vi "Utility - Build VIHelpeks Help and Link to VIs.vi"() -> ()   [LabVIEW 2014]
doc: "::: VI Helpeks :::\nCopyright (c) 2000-2026 Konstantin Shifershteyn. All rights reserved."
uses:
  <vilib>/Platform/browser.llb/Open URL in Default Browser (path).vi
  vi.lib/addons/VI Helpeks/VIHelpeksAPI.lvlib
panel:
  out "VI Help Info":T1(array[cluster])
  out "error out":errorcluster
  in  "Save Params":T2
  in  "Build Params":T3={"Help Targeting"=enum."<helpdir>", "Subfolder"="VI Helpeks", "CHM Tag mode"=enum."HTML Filename"}
  out "Errors":i32
  out "Paths":T4
  in  "Generate CHM (T)":bool=TRUE
  in  "Show Progress Window (T)":bool=TRUE
  in  "VIHelpeks Project File":path=path "../Help Project/VIHelpeks.hgprj"
  # "VI Helpeks\nCopyright (c) 2012-2026 Konstantin Shifershteyn"
  # "Apply Help Configuration to VIs"
  # "Generate Help"
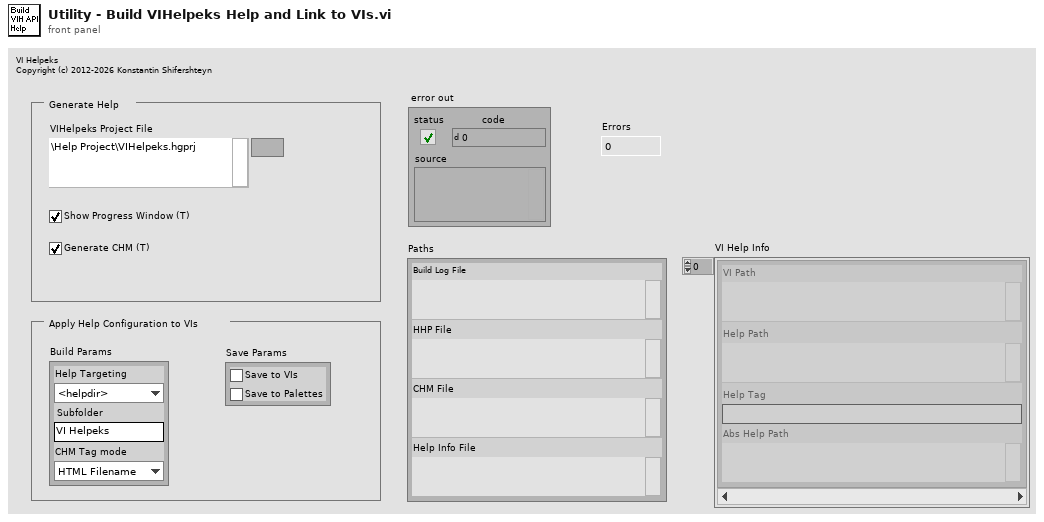
[diagram p1: front panel]
types:
  T1 = cluster{"VI Path":path, "Help Path":path, "Help Tag":string, "Abs Help Path":path}[]
  T2 = cluster{"Save to VIs":bool, "Save to Palettes":bool}
  T3 = cluster{"Help Targeting":enum16{"absolute", "relative", "<helpdir>", "<userlib>", "<vilib>", "<instrlib>"}, "Subfolder":string, "CHM Tag mode":enum16{"HTML Filename", "Index Keyword"}}
  T4 = cluster{"Build Log File":path, "HHP File":path, "CHM File":path, "Help Info File":path}
  T5 = cluster{"Help Path":path, "Help Tag":string, "Abs Help Path":path}[]
  T6 = cluster{"Original File Path":path, "Help Path":path, "Help Tag":string, "Abs Help Path":path}
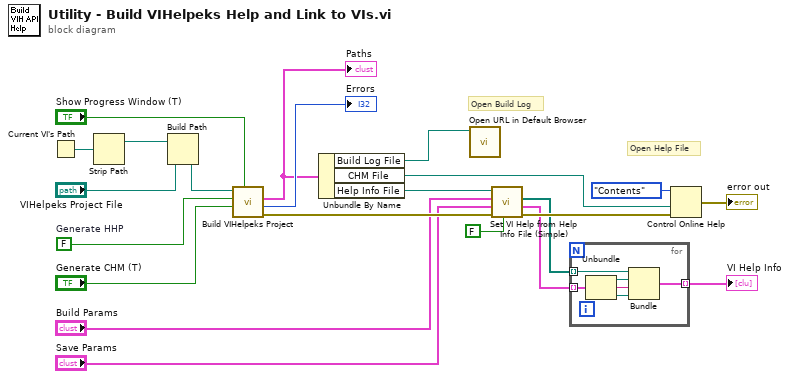
[diagram p0: block diagram]
diagram:
  w21 = FALSE  # Generate HHP
  # "Open Help File"
  # "Open Build Log"
  n1 = Current VI's Path() -> (path=w4:path)
  n2 = Strip Path(path=w4) -> (stripped path=w3:path)  [unwired: 1 out]
  n3 = Build Path(base path=w3, name or relative path="VIHelpeks Project File") -> (appended path=w1:path)
  n4 = call "Build VIHelpeks Project.vi"("Show Progress Window (T)"="Show Progress Window (T)", "Generate CHM (T)"="Generate CHM (T)", "Generate HHP (T)"=w21, "VIHelpeks Project File"=w1) -> ("error out"=w18:errorcluster, "Errors"=→"Errors":i32, "Paths"=w15:T4)  [unwired: 4 in, 1 out]
  "Paths" <- w15
  n5 = Unbundle By Name(w15) -> ("Build Log File"=w12:path, "CHM File"=w11:path, "Help Info File"=w14:path)
  n6 = call-poly <vilib>:"Open URL in Default Browser.vi"("path"=w12) -> ()  [unwired: 5 in, 2 out]
  n7 = call "Set VI Help from Help Info File (Simple).vi"("Link to HTML (F)"=FALSE, "error in"=w18, "Save Params"="Save Params", "Build Params"="Build Params", "Help Info File"=w14) -> ("error out"=w10:errorcluster, "Source Files Help Info"=w7:T5, "Source File Paths"=w6:path[])  [unwired: 3 in, 1 out]
  n8 = for {
    tunnel: w7 -> [w28] mode=indexing
    tunnel: w6 -> [w27] mode=indexing
    tunnel: [w24] -> w5 mode=indexing
    n9 = Unbundle(w28) -> ("Help Path"=w26:path, "Help Tag"=w25:string, "Abs Help Path"=w23:path)
    n10 = Bundle("Original File Path"=w27, "Help Path"=w26, "Help Tag"=w25, "Abs Help Path"=w23) -> (w24:T6)  [unwired: 1 in]
  }
  "VI Help Info" <- w5
  n11 = Control Online Help(1:w10, 2:w11, 4:enum16{"Contents", "Key", "Close"}."Contents" ("Operation")) -> (0:→"error out":errorcluster)  [unwired: 1 in]
